vi "Pirani_V_to_Pa.vi"(0 "V_in":dbl) -> (1 "P_Pa":dbl, 2 "P_mbar":dbl, 3 "Sensor_fault":bool, 4 "At_atm":bool)   [LabVIEW 2025]
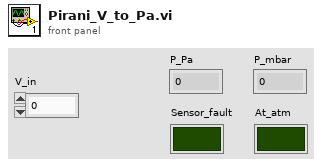
[diagram p1: front panel]
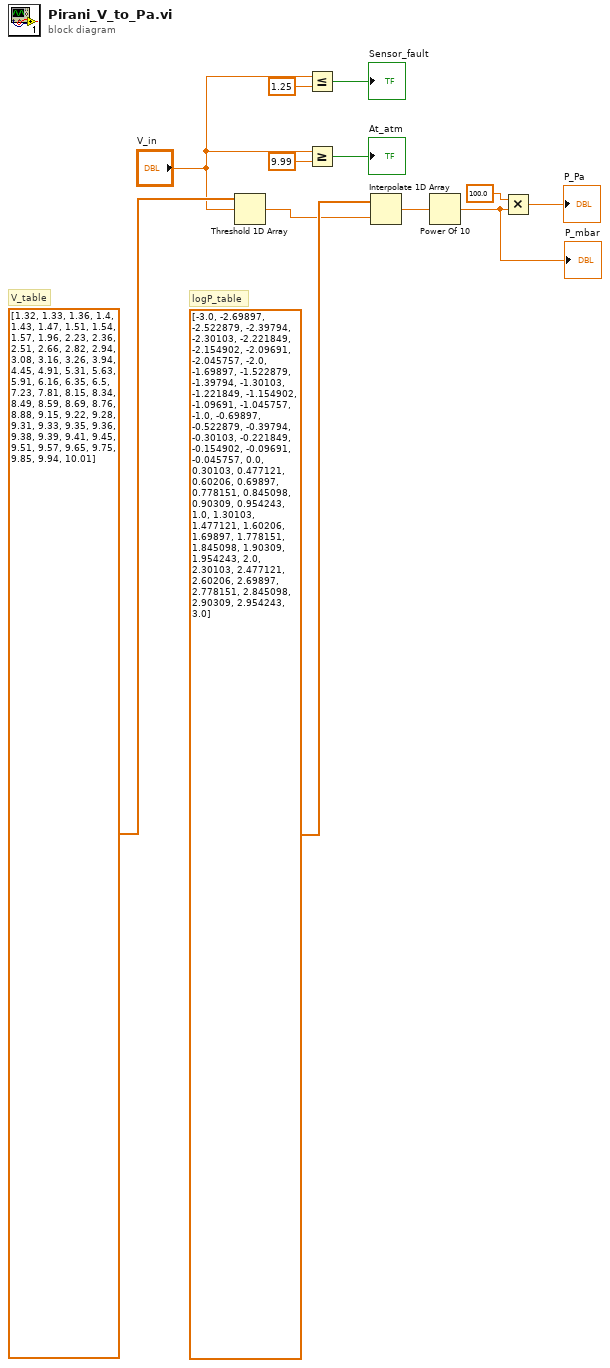
[diagram p0: block diagram]
diagram:
  # "logP_table"
  # "V_table"
  n1 = Threshold 1D Array(2:"V_in", 3:dbl[] [1.32, 1.33, 1.36, 1.4, 1.43, 1.47, 1.51, 1.54, 1.57, 1.96, 2.23, 2.36, 2.51, 2.66, 2.82, 2.94, 3.08, 3.16, 3.26, 3.94, 4.45, 4.91, 5.31, 5.63, 5.91, 6.16, 6.35, 6.5, 7.23, 7.81, 8.15, 8.34, 8.49, 8.59, 8.69, 8.76, 8.88, 9.15, 9.22, 9.28, 9.31, 9.33, 9.35, 9.36, 9.38, 9.39, 9.41, 9.45, 9.51, 9.57, 9.65, 9.75, 9.85, 9.94, 10.01]) -> (0:w10:dbl)  [unwired: 1 in]
  n2 = Less Or Equal?(x="V_in", y=1.25) -> (x <= y?=→"Sensor_fault":bool)
  n3 = Greater Or Equal?(x="V_in", y=9.99) -> (x >= y?=→"At_atm":bool)
  n4 = Interpolate 1D Array(1:w10, 2:dbl[] [-3.0, -2.69897, -2.522879, -2.39794, -2.30103, -2.221849, -2.154902, -2.09691, -2.045757, -2.0, -1.69897, -1.522879, -1.39794, -1.30103, -1.221849, -1.154902, -1.09691, -1.045757, -1.0, -0.69897, -0.522879, -0.39794, -0.30103, -0.221849, -0.154902, -0.09691, -0.045757, 0.0, 0.30103, 0.477121, 0.60206, 0.69897, 0.778151, 0.845098, 0.90309, 0.954243, 1.0, 1.30103, 1.477121, 1.60206, 1.69897, 1.778151, 1.845098, 1.90309, 1.954243, 2.0, 2.30103, 2.477121, 2.60206, 2.69897, 2.778151, 2.845098, 2.90309, 2.954243, 3.0]) -> (0:w9:dbl)
  n5 = Power Of 10(x=w9) -> (10^x=w1:dbl)
  "P_mbar" <- w1
  n6 = Multiply(x=100.0, y=w1) -> (x*y=→"P_Pa":dbl)
